vi "Blank VI 01.vi"(7 "Calling VI Ref":refnum<vi>) -> ()   [LabVIEW 2016]
uses:
  <vilib>/Utility/miscctls.llb/LVPointTypeDef.ctl
panel:
  out "Right":i16
  out "Bottom":i16
  in  "Quit":bool
  out "Numeric":i32
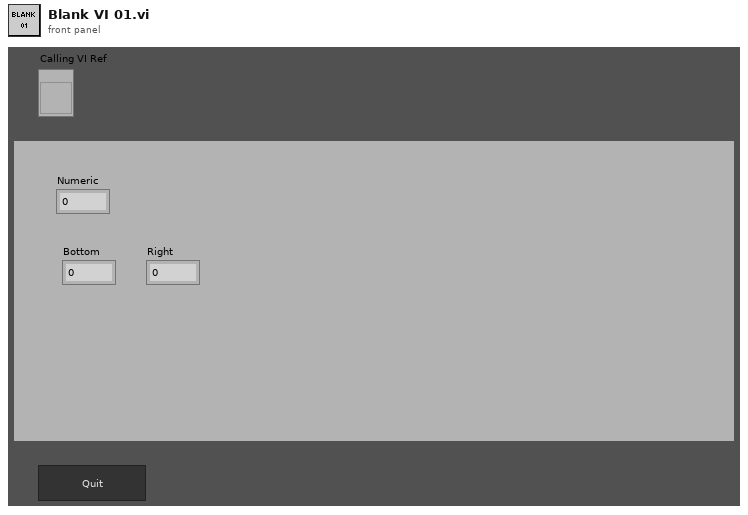
[diagram p1: front panel]
types:
  T1 = enum16{"Always On", "Always Off", "Off While Running"}
  T2 = typedef "LVPointTypeDef.ctl" = cluster{"Horizontal":i16, "Vertical":i16}
  T3 = typedef "LVRectTypeDef.ctl" = cluster{"Left":i16, "Top":i16, "Right":i16, "Bottom":i16}
  T4 = typedef "LVBoundsTypeDef.ctl" = cluster{"Width":u32, "Height":u32}
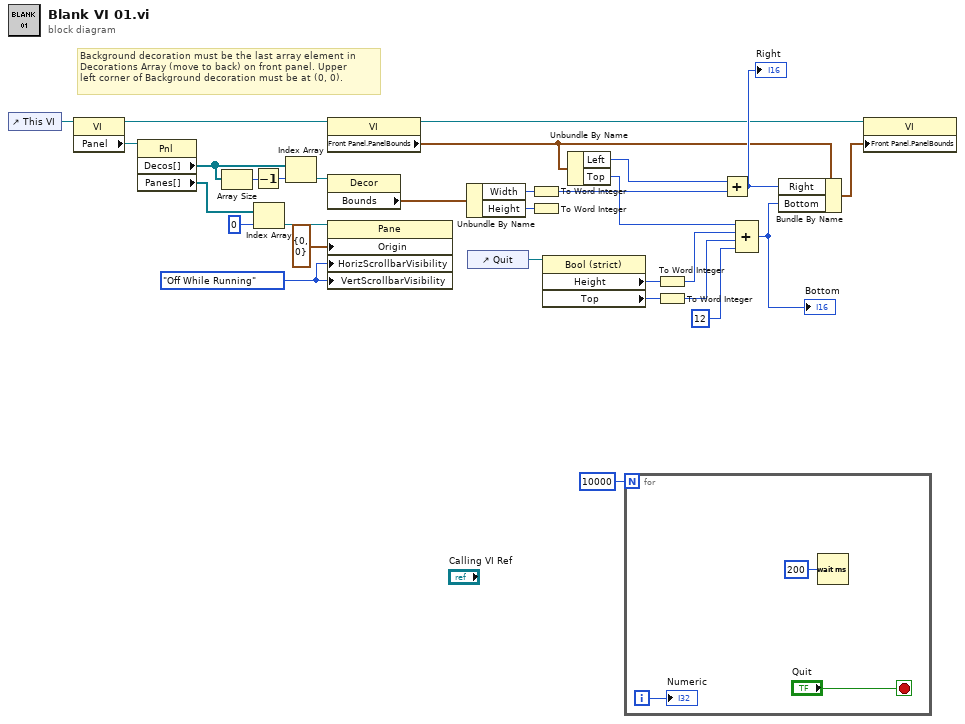
[diagram p0: block diagram]
diagram:
  w12 = T1."Off While Running" ("Vertical Scrollbar Visibility")
  # "Background decoration must be the last array element in\nDecorations Array (move to back) on front panel. Upper\nleft corner of Background decoration must be at (0, 0)."
  n1 = control-ref of="This VI"() -> (w5:refnum<vi>)
  n2 = property class="VI"(reference=w5) -> (reference out=w13:refnum<vi>, "Panel"=w6:refnum<vi>)  [unwired: 1 in, 1 out]
  n3 = property class="Pnl"(reference=w6) -> ("Decos[]"=w4:refnum<vi>[], "Panes[]"=w9:refnum<vi>[])  [unwired: 1 in, 2 out]
  n4 = Array Size(array=w4) -> (size(s)=w2:i32)
  n5 = Decrement(x=w2) -> (x-1=w3:i32)
  n6 = Index Array(array=w9, index=0) -> (element=w8:refnum<vi>)
  n7 = Index Array(array=w4, index=w3) -> (element=w11:refnum<vi>)
  n8 = property class="VI"(reference=w13) -> (reference out=w15:refnum<vi>, "Front Panel.PanelBounds"=w16:T3)  [unwired: 1 in, 1 out]
  n9 = property class="Decor"(reference=w11) -> ("Bounds"=w14:T4)  [unwired: 1 in, 2 out]
  n10 = property class="Pane"(reference=w8, "Origin"=T2 {"Horizontal"=0, "Vertical"=0}, "HorizScrollbarVisibility"=w12, "VertScrollbarVisibility"=w12) -> ()  [unwired: 1 in, 2 out]
  n11 = Unbundle By Name(w14) -> ("Width"=w19:u32, "Height"=w22:u32)
  n12 = control-ref of="Quit"() -> (w1:refnum<vi>)
  n13 = To Word Integer(number=w19) -> (16bit integer=w21:i16)
  n14 = To Word Integer(number=w22) -> ()  [unwired: 1 out]
  n15 = property class="Bool (strict)"(reference=w1) -> ("Height"=w24:u32, "Top"=w25:i32)  [unwired: 1 in, 2 out]
  n16 = Unbundle By Name(w16) -> ("Left"=w18:i16, "Top"=w29:i16)
  n17 = for {
    N: 10000 -> [_]
    i -> [w32]
    stop <- "Quit" stop-if-true
    n18 = Wait (ms)(milliseconds to wait=u32 200) -> ()  [unwired: 1 out]
    "Numeric" <- w32
  }
  n19 = To Word Integer(number=w24) -> (16bit integer=w27:i16)
  n20 = To Word Integer(number=w25) -> (16bit integer=w28:i16)
  n21 = Add(x=w18, y=w21) -> (x+y=w20:i16)
  "Right" <- w20
  n22 = Compound Arithmetic op=ADD(w29, w27, w28, i16 12 ("y")) -> (w23:i16)
  "Bottom" <- w23
  n23 = Bundle By Name(cluster=w16, "Right"=w20, "Bottom"=w23) -> (w17:T3)
  n24 = property class="VI"(reference=w15, "Front Panel.PanelBounds"=w17) -> ()  [unwired: 1 in, 2 out]
